vi "Inst_Open.vi"(8 "error in (no error)":errorcluster, 10 "TermChar":u8=10, 11 "VISA Refnum in":refnum<visa-resource-name>) -> (0 "error out":errorcluster, 3 "VISA Refnum out":refnum<visa-resource-name>)   [LabVIEW 2018]
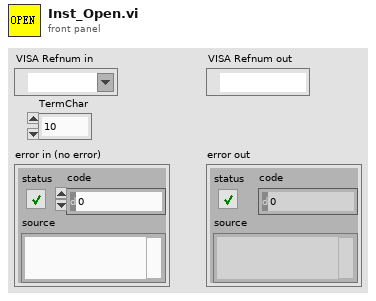
[diagram p1: front panel]
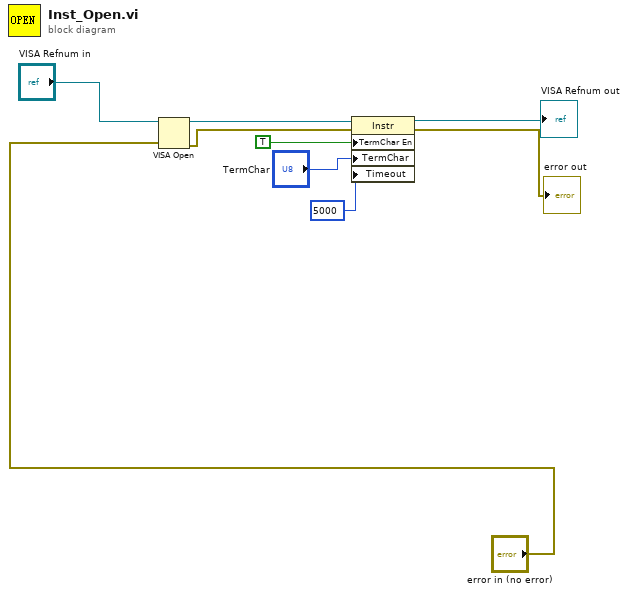
[diagram p0: block diagram]
diagram:
  n1 = VISA Open(error in (no error)="error in (no error)", VISA resource name="VISA Refnum in") -> (VISA resource name=w3:refnum<visa-resource-name>, error out=w6:errorcluster)  [unwired: 3 in]
  n2 = property class="Instr"(reference=w3, error in=w6, "TermChar En"=TRUE ("Message Based Settings:Termination Character Enable"), "TermChar"="TermChar", "Timeout"=u32 5000 ("General Settings:Timeout Value")) -> (reference out=→"VISA Refnum out":refnum<visa-resource-name>, error out=→"error out":errorcluster)
